vi "Cursor Move.vi"(8 "error in (no error)":errorcluster, 9 "Active Plot":i32, 10 "CursLocation":cluster{"X":dbl, "Y":dbl}, 11 "UI Refs":T1) -> (0 "error out":errorcluster)   [LabVIEW 2025, in "XY Plotter.lvlib" / "XY Plotter.lvclass"]
uses:
  XY Plotter.lvclass
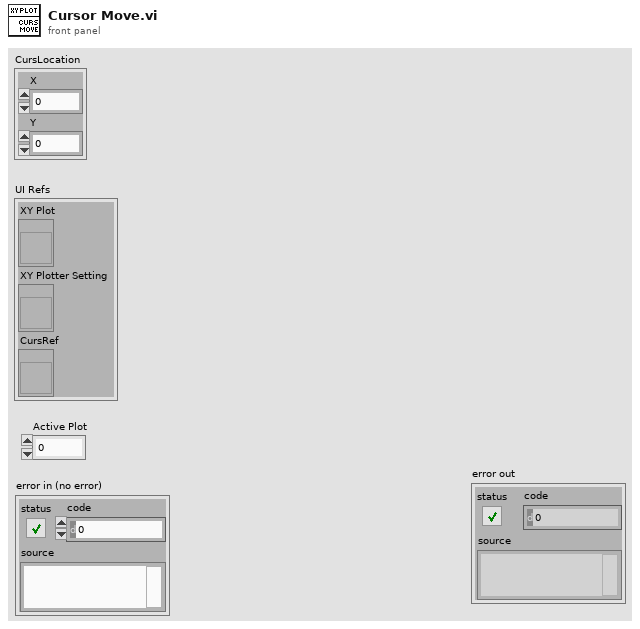
[diagram p1: front panel]
types:
  T1 = cluster{"XY Plot":refnum<vi>, "XY Plotter Setting":refnum<vi>, "CursRef":refnum<vi>}
  T2 = typedef "LVPoint32TypeDef.ctl" = cluster{"Horizontal":i32, "Vertical":i32}
  T3 = typedef "XY Plotter.lvlib/XY Plotter configuration.lvclass/XY Plotter.ctl" = cluster{"Data Rate":i32, "Y-Scales":cluster{"Label":string, "Max":dbl, "Min":dbl, "Unit":enum16{"---", "V", "mA", "sec", "dB", "deg", "in/s", "in", "lbf", "Hz", "psi", "gpm"}, "Visible":bool}[], "Note":string, "History Length":i32, "DataLog Path":path, "Plot type":bool, "X-Scales":cluster{"Label":string, "Max":dbl, "Min":dbl, "Unit":enum16{"---", "V", "mA", "sec", "dB", "deg", "in/s", "in", "lbf", "Hz", "psi", "gpm"}, "Visible":bool}[], "Plot List":cluster{"Plot Name":string, "X Scale Index":u32, "Y Scale Index":u32, "Visible":bool}[]}
  T4 = cluster{"Label":string, "Max":dbl, "Min":dbl, "Unit":enum16{"---", "V", "mA", "sec", "dB", "deg", "in/s", "in", "lbf", "Hz", "psi", "gpm"}, "Visible":bool}[]
  T5 = cluster{"Plot Name":string, "X Scale Index":u32, "Y Scale Index":u32, "Visible":bool}[]
  T6 = typedef "LVRectTypeDef.ctl" = cluster{"Left":i16, "Top":i16, "Right":i16, "Bottom":i16}
  T7 = cluster{"Plot Name":string, "X Scale Index":u32, "Y Scale Index":u32, "Visible":bool}
  T8 = cluster{"Label":string, "Max":dbl, "Min":dbl, "Unit":enum16{"---", "V", "mA", "sec", "dB", "deg", "in/s", "in", "lbf", "Hz", "psi", "gpm"}, "Visible":bool}
  T9 = enum16{"---", "V", "mA", "sec", "dB", "deg", "in/s", "in", "lbf", "Hz", "psi", "gpm"}
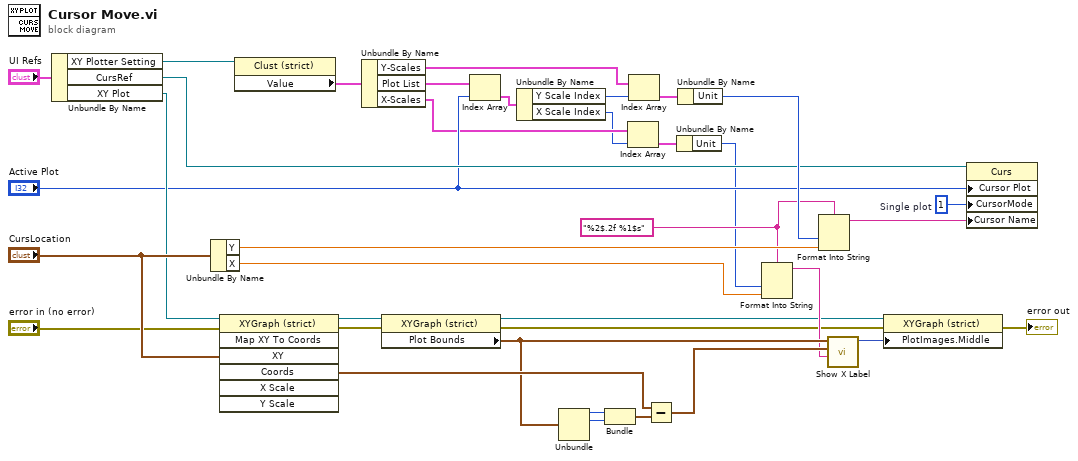
[diagram p0: block diagram]
diagram:
  w5 = "%2$.2f %1$s" ("format string")
  w30 = u32 1  # Single plot
  n1 = Unbundle By Name("UI Refs") -> ("XY Plotter Setting"=w17:refnum<vi>, "CursRef"=w14:refnum<vi>, "XY Plot"=w9:refnum<vi>)
  n2 = Unbundle By Name("CursLocation") -> ("Y"=w32:dbl, "X"=w33:dbl)
  n3 = invoke on="Invoke Node" class="XYGraph (strict)" method="Map XY To Coords"(reference=w9, error in="error in (no error)", "XY"="CursLocation") -> (reference out=w26:refnum<vi>, error out=w12:errorcluster, "Coords"=w27:T2)  [unwired: 4 in, 4 out]
  n4 = property class="Clust (strict)"(reference=w17) -> ("Value"=w28:T3)  [unwired: 1 in, 2 out]
  n5 = Unbundle By Name(w28) -> ("Y-Scales"=w7:T4, "Plot List"=w34:T5, "X-Scales"=w4:T4)
  n6 = property class="XYGraph (strict)"(reference=w26, error in=w12) -> (reference out=w18:refnum<vi>, error out=w11:errorcluster, "Plot Bounds"=w23:T6)
  n7 = Index Array(array=w34, index="Active Plot") -> (element=w35:T7)
  n8 = Unbundle By Name(w35) -> ("Y Scale Index"=w36:u32, "X Scale Index"=w3:u32)
  n9 = Unbundle(w23) -> ("Left"=w22:i16, "Top"=w21:i16)  [unwired: 2 out]
  n10 = Bundle("Left"=w22, "Top"=w21) -> (w24:cluster{"Left":i16, "Top":i16})  [unwired: 1 in]
  n11 = Index Array(array=w4, index=w3) -> (element=w2:T8)
  n12 = Index Array(array=w7, index=w36) -> (element=w29:T8)
  n13 = Subtract(x=w27, y=w24) -> (x-y=w25:T2)
  n14 = Unbundle By Name(w2) -> ("Unit"=w1:T9)
  n15 = Unbundle By Name(w29) -> ("Unit"=w31:T9)
  n16 = Format Into String(format string=w5, w1, w33) -> (resulting string=w20:string)  [unwired: 2 in, 1 out]
  n17 = Format Into String(format string=w5, w31, w32) -> (resulting string=w6:string)  [unwired: 2 in, 1 out]
  n18 = call "Show X Label.vi"("String"=w20, "pixel center"=w25, "Rect"=w23) -> ("new picture out"=w19:picture)  [unwired: 7 in, 1 out]
  n19 = property class="XYGraph (strict)"(reference=w18, error in=w11, "PlotImages.Middle"=w19) -> (error out=→"error out":errorcluster)  [unwired: 1 out]
  n20 = property class="Curs"(reference=w14, "Cursor Plot"="Active Plot", "CursorMode"=w30, "Cursor Name"=w6) -> ()  [unwired: 1 in, 2 out]
